vi "Timer_Reset.vi"(8 "Pass_Through_Time":dbl=-1.0 format="%33.4f", 11 "in TIMER":T1 {"Accumulated TIme" format="%13.5p"; "StartTime" format="%13.5p"}) -> (3 "out TIMER":T1 {"Accumulated TIme" format="%13.5p"; "StartTime" format="%13.5p"})   [LabVIEW 2019, in "Trajectory_Library.lvlib"]
doc: "Reset the timer by setting the time to 0. Make the timer startTime the current time so new requests will be relative now\n\nInputs:\n - Timer -- The Timer data cluster\n\nOutputs:\n - Timer -- The modified Timer data cluster"
uses:
  Trajectory_Library.lvlib
  TypeDef/TIMER.ctl
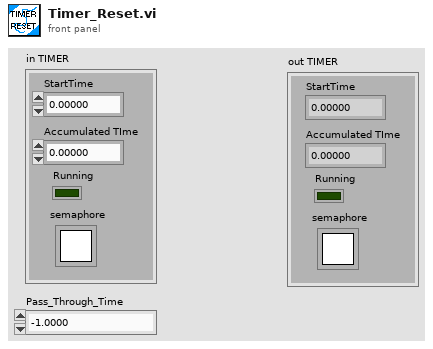
[diagram p1: front panel]
types:
  T1 = typedef "Trajectory_Library.lvlib/TIMER.ctl" = cluster{"StartTime":dbl, "Accumulated TIme":dbl, "Running":bool, "semaphore":T2}
  T2 = typedef "Semaphore RefNum" = refnum<k1>
  T3 = typedef "WPILib_Math.lvlib/TIMER.ctl" = cluster{"StartTime":dbl, "Accumulated TIme":dbl, "Running":bool, "semaphore":T2}
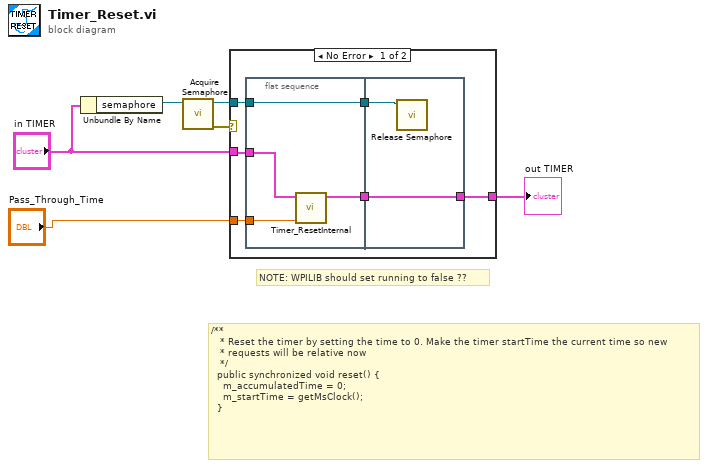
[diagram p0: block diagram]
diagram:
  # "NOTE: WPILIB should set running to false ??"
  # "/**\n   * Reset the timer by setting the time to 0. Make the timer startTime the current time so new\n   * requests will be relative now\n   */\n  public synchronized void reset() {\n    m_accumulatedTime = 0;\n    m_startTime = getMsClock();\n  }"
  n1 = Unbundle By Name("in TIMER") -> ("semaphore"=w5:T2)
  n2 = call <vilib>:"Acquire Semaphore.vi"("semaphore"=w5) -> ("error out"=w4:errorcluster, "semaphore out"=w2:T2)  [unwired: 4 in, 1 out]
  n3 = case shown="No Error" w4 {
    tunnel: [w12 w19] -> w6
    tunnel: "in TIMER" -> [w11 w19]
    tunnel: w2 -> [w8 _]
    tunnel: "Pass_Through_Time" -> [w7 _]
    frame No Error {
      n4 = flat-sequence {
        tunnel: w11 -> [w15]
        tunnel: [w16] -> w10
        tunnel: [w14] -> w9
        tunnel: w8 -> [w14]
        tunnel: w7 -> [w13]
        tunnel: [w18] -> w12
        tunnel: w10 -> [w18]
        tunnel: w9 -> [w17]
        frame #0 {
          n5 = call "Timer_ResetInternal.vi"("Pass_Through_Time"=w13, "in TIMER"=w15) -> ("out TIMER"=w16:T3)  [unwired: 9 in]
        }
        frame #1 {
          n6 = call <vilib>:"Release Semaphore.vi"("semaphore"=w17) -> ()  [unwired: 5 in, 2 out]
        }
      }
    }
    frame Error {
    }
  }
  "out TIMER" <- w6
